vi "Send Precision Response.vi"(8 "error in (no error)":errorcluster caption="에러 입력(에러 없음)", 9 "Amplitude":dbl, 10 "id":string, 11 "Instrument Manager 입력":refnum<class "Instrument Manager.lvclass">) -> (0 "error out":errorcluster caption="에러 출력", 3 "Instrument Manager 출력":refnum<class "Instrument Manager.lvclass">)   [LabVIEW 2023, in "Instrument Manager.lvclass"]
uses:
  Instrument Manager.lvclass
  Instrument Manager.lvclass/Instrument Manager.ctl
  Precision Response.ctl
  Error Response.ctl
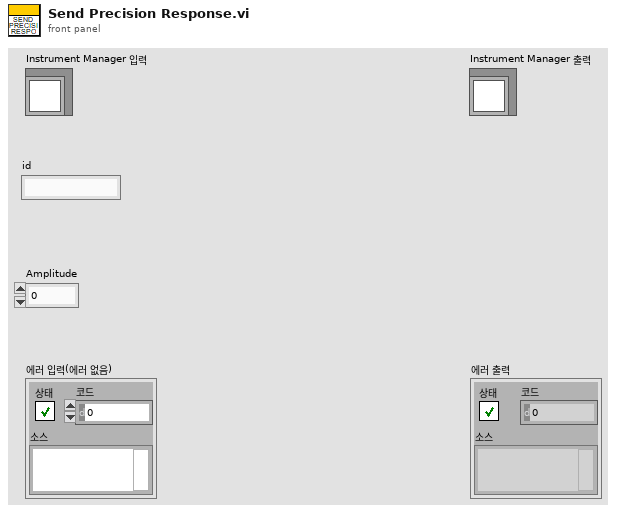
[diagram p1: front panel]
types:
  T1 = typedef "Instrument Manager.lvclass/Precision Response.ctl" = cluster{"type":string, "id":string, "status":string, "Result":cluster{"Amplitude":dbl}}
  T2 = cluster{"Reader Q":refnum<queue>, "Writer Q":refnum<queue>}
  T3 = typedef "Instrument Manager.lvclass/Error Response.ctl" = cluster{"type":string, "id":string, "status":string, "error out":errorcluster}
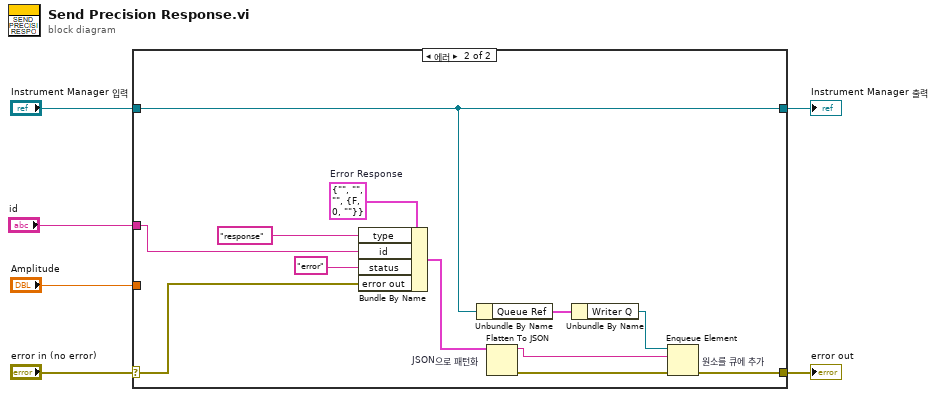
[diagram p0: block diagram]
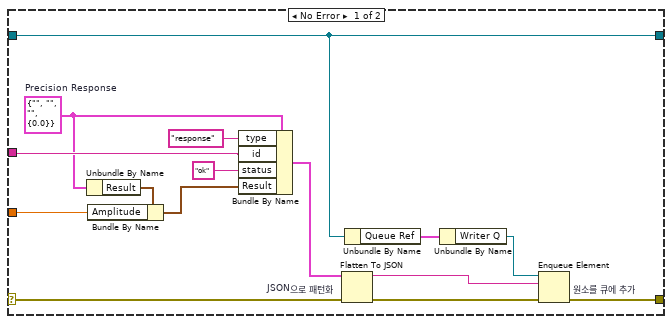
[diagram p2: hidden frame]
diagram:
  n1 = case shown="에러" "error in (no error)" {
    selector: "error in (no error)" -> [w15 w24]
    tunnel: [w8 w23] -> w5
    tunnel: [w11 w25] -> w3
    tunnel: "Instrument Manager 입력" -> [w11 w25]
    tunnel: "id" -> [w17 w22]
    tunnel: "Amplitude" -> [w16 _]
    frame No Error {
      w14 = T1 {"type"="", "id"="", "status"="", "Result"={"Amplitude"=0.0}}  # Precision Response
      n2 = Unbundle By Name(w14) -> ("Result"=w19:cluster{"Amplitude":dbl})
      n3 = Bundle By Name(cluster=w19, "Amplitude"=w16) -> (w18:cluster{"Amplitude":dbl})
      n4 = Bundle By Name(cluster=w14, "type"="response", "id"=w17, "status"="ok", "Result"=w18) -> (w13:T1)
      n5 = Flatten To JSON "JSON으로 패턴화"(anything=w13, error in (no error)=w15) -> (JSON string=w7:string, 11:w9:errorcluster)  [unwired: 1 in]
      n6 = Unbundle By Name(w11) -> ("Queue Ref"=w12:T2)
      n7 = Unbundle By Name(w12) -> ("Writer Q"=w10:refnum<queue>)
      n8 = Enqueue Element "원소를 큐에 추가"(queue=w10, element=w7, error in (no error)=w9) -> (error out=w8:errorcluster)  [unwired: 1 in, 2 out]
    }
    frame Error {
      w33 = T3 {"type"="", "id"="", "status"="", "error out"={"status"=FALSE, "code"=0, "source"=""}}  # Error Response
      n9 = Bundle By Name(cluster=w33, "type"="response", "id"=w22, "status"="error", "error out"=w24) -> (w29:T3)
      n10 = Unbundle By Name(w25) -> ("Queue Ref"=w27:T2)
      n11 = Flatten To JSON "JSON으로 패턴화"(anything=w29) -> (JSON string=w32:string, 11:w28:errorcluster)  [unwired: 2 in]
      n12 = Unbundle By Name(w27) -> ("Writer Q"=w26:refnum<queue>)
      n13 = Enqueue Element "원소를 큐에 추가"(queue=w26, element=w32, error in (no error)=w28) -> (error out=w23:errorcluster)  [unwired: 1 in, 2 out]
    }
  }
  "error out" <- w5
  "Instrument Manager 출력" <- w3
